vi "Init with Values.vi"(8 "error in":errorcluster, 10 "Values":variant, 11 "Combo Box in":refnum<class "Combo Box.lvclass">) -> (0 "error out":errorcluster, 3 "Combo Box out":refnum<class "Combo Box.lvclass">)   [LabVIEW 2020, in "SourceGrid.lvlib" / "Combo Box.lvclass"]
doc: "Values: ICollection compatible set of standard values"
uses:
  Combo Box.lvclass
  Combo Box.lvclass/Combo Box.ctl
  D:/git/Sourcegrid-LabVIEW/source/SourceGrid.dll
  SourceGrid.dll
  <vilib>/Utility/Data Type/NI_Data Type.lvlib
  <vilib>/Platform/dotnet.llb/To .NET Framework Object.vi
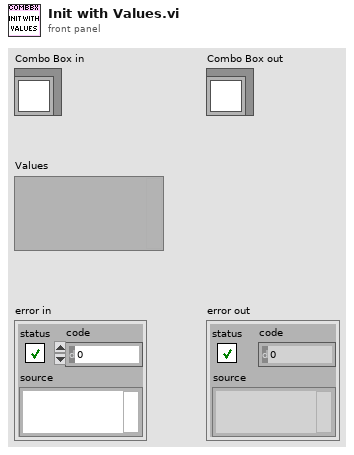
[diagram p1: front panel]
types:
  T1 = typedef "NI_Data Type.lvlib/Data Type.ctl" = enum8{"Invalid Type", "Void", "I8", "I16", "I32", "I64", "U8", "U16", "U32", "U64", "Single Float", "Double Float", "Extended Float", "Single Complex", "Double Complex", "Extended Complex", "Enum U8", "Enum U16", "Enum U32", "Enum U64", "Single Float With Unit", "Double Float With Unit", "Extended Float With Unit", "Single Complex with Unit", "Double Complex with Unit", "Extended Complex with Unit", "Boolean", "String", "Path", "Picture", "Tag", "Array", "Cluster", "Variant", "LV Variant", "Waveform", "Timestamp", "Digital Waveform", "Digital Data", "ExpressData", "Refnum", "External Data", "VI", "Poly VI", "LabVIEW Class Instance", "Fixed Point", "Set Collection", "Map Collection"}
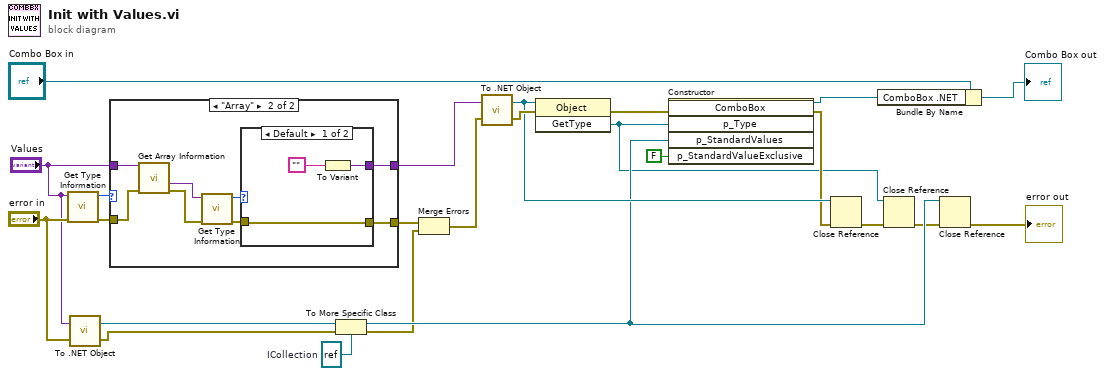
[diagram p0: block diagram]
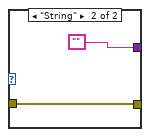
[diagram p3: hidden frame]
diagram:
  w17 = refnum<k24> refnum  # ICollection
  n1 = call <vilib>:"Get Type Information.vi"("error in (no error)"="error in", "variant"="Values") -> ("error out"=w23:errorcluster, "type"=w24:T1)  [unwired: 5 in, 3 out]
  n2 = call-poly <vilib>:"To .NET Object.vi"("error in (no error)"="error in", "anything"="Values") -> ("error out"=w9:errorcluster, ".NET object"=w20:refnum<k24>)
  n3 = case shown="\"Array\"" w24 {
    tunnel: w23 -> [w26 w32]
    tunnel: "Values" -> [w25 w34]
    tunnel: [w25 w28] -> w22
    tunnel: [w26 w27] -> w10
    frame Default {
    }
    frame "Array" {
      n4 = call <vilib>:"Get Array Information.vi"("error in (no error)"=w32, "variant"=w34) -> ("error out"=w31:errorcluster, "array element data type"=w29:variant)  [unwired: 6 in, 2 out]
      n5 = call <vilib>:"Get Type Information.vi"("error in (no error)"=w31, "variant"=w29) -> ("error out"=w30:errorcluster, "type"=w33:T1)  [unwired: 5 in, 3 out]
      n6 = case shown="Default" w33 {
        tunnel: w30 -> [w37 w39]
        tunnel: [w37 w39] -> w27
        tunnel: [w35 ""] -> w28
        frame Default {
          n7 = To Variant(anything="") -> (Variant=w35:variant)
        }
        frame "String" {
        }
      }
    }
  }
  n8 = To More Specific Class(target class=w17, reference=w20, error in=w9) -> (specific class reference=w7:refnum<k24>, error out=w5:errorcluster)
  n9 = Merge Errors(w10, w5) -> (w6:errorcluster)
  n10 = call-poly <vilib>:"To .NET Object.vi"("error in (no error)"=w6, "anything"=w22) -> ("error out"=w21:errorcluster, ".NET object"=w11:refnum<k24>)
  n11 = invoke class="Object" method="GetType"(reference=w11, error in=w21) -> (error out=w15:errorcluster, "GetType"=w1:refnum<k24>)  [unwired: 1 in, 1 out]
  n12 = constructor class="ComboBox"(error in=w15, "p_Type"=w1, "p_StandardValues"=w7, "p_StandardValueExclusive"=FALSE) -> (reference out=w3:refnum<k24>, error out=w4:errorcluster)  [unwired: 2 in, 4 out]
  n13 = Close Reference(reference=w11, error in (no error)=w4) -> (error out=w12:errorcluster)
  n14 = Bundle By Name(cluster="Combo Box in", "ComboBox .NET"=w3) -> (→"Combo Box out":refnum<class "Combo Box.lvclass">)
  n15 = Close Reference(reference=w1, error in (no error)=w12) -> (error out=w2:errorcluster)
  n16 = Close Reference(reference=w7, error in (no error)=w2) -> (error out=→"error out":errorcluster)
